vi "Disconnect.vi"(8 "error in (no error)":errorcluster, 11 "ImageHandler:DT-ImageHandler in":refnum<class "DT-ImageHandler.lvclass">) -> (0 "error out":errorcluster, 3 "ImageHandler:DT-ImageHandler out":refnum<class "DT-ImageHandler.lvclass">)   [LabVIEW 2022 SP3, in "ImageHandler.lvlib" / "DT-ImageHandler.lvclass"]
uses:
  DT-ImageHandler.lvclass
  DT-ImageHandler.lvclass/DT-ImageHandler.ctl
  xPanelWrapperLvLib/xPanelWrapper.lvlib
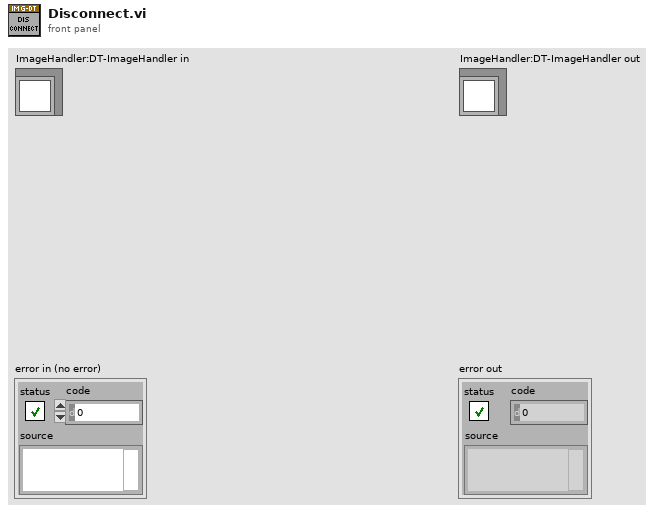
[diagram p1: front panel]
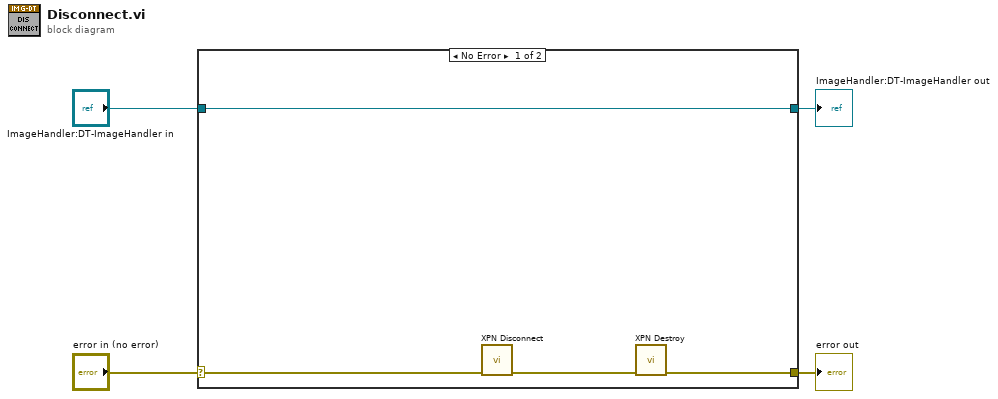
[diagram p0: block diagram]
diagram:
  n1 = case shown="No Error" "error in (no error)" {
    selector: "error in (no error)" -> [w7 w10]
    tunnel: [w5 w10] -> w3
    tunnel: [w8 w9] -> w1
    tunnel: "ImageHandler:DT-ImageHandler in" -> [w8 w9]
    frame No Error {
      n2 = call "XPN Disconnect.vi"("error in (no error)"=w7) -> ("error out"=w6:errorcluster)  [unwired: 9 in, 1 out]
      n3 = call "XPN Destroy.vi"("error in (no error)"=w6) -> ("error out"=w5:errorcluster)  [unwired: 9 in, 1 out]
    }
    frame Error {
    }
  }
  "error out" <- w3
  "ImageHandler:DT-ImageHandler out" <- w1
